vi "log.vi"(8 "error in (no error)":errorcluster, 10 "log_entry":T1 {"datetime" format="%<%x %.3X>T"}, 11 "system.logging.provider in":refnum<class "system.logging.provider.lvclass">) -> (0 "error out":errorcluster, 3 "system.logging.provider out":refnum<class "system.logging.provider.lvclass">)   [LabVIEW 2021, in "system.logging.provider.lvclass"]
uses:
  system.logging.provider.lvclass
  system.logging/log_entry.ctl
  system.logging/severity.ctl
  system.logging.provider.lvclass/system.logging.provider.ctl
  system.logging/system.logging.lvclass
panel:
  out "log_entry_display":T1 {"datetime" format="%<%x %.3X>T"}
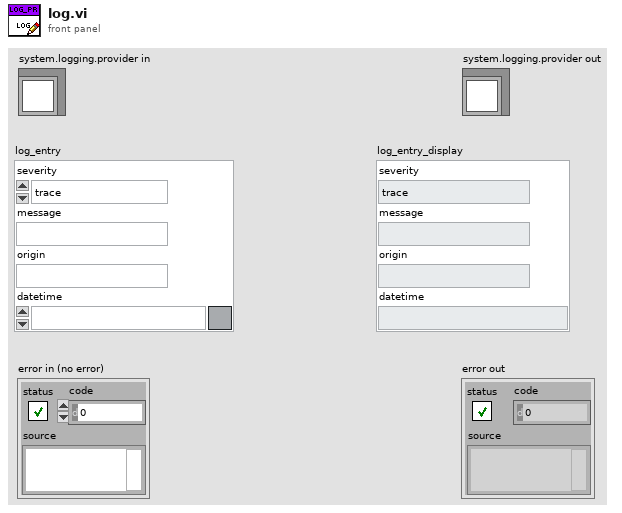
[diagram p1: front panel]
types:
  T1 = typedef "system.logging.lvclass/log_entry.ctl" = cluster{"severity":T2, "message":string, "origin":string, "datetime":timestamp}
  T2 = typedef "system.logging.lvclass/severity.ctl" = enum8{"trace", "debug", "info", "warning", "error"}
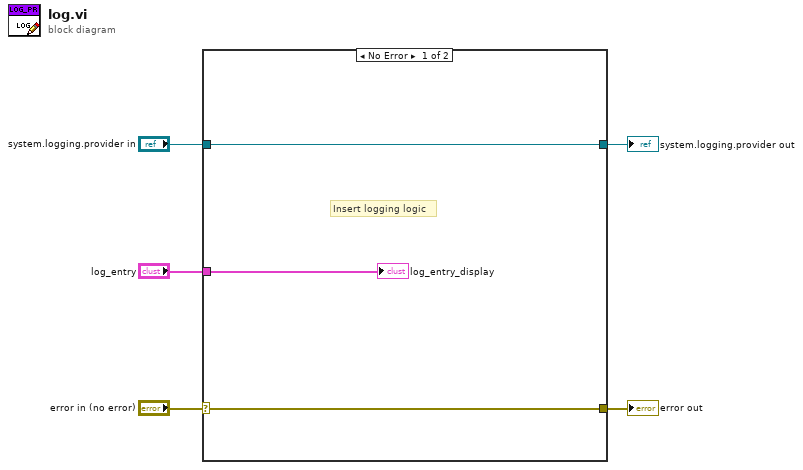
[diagram p0: block diagram]
diagram:
  n1 = case shown="No Error" "error in (no error)" {
    selector: "error in (no error)" -> [w7 w10]
    tunnel: [w7 w10] -> w4
    tunnel: [w6 w9] -> w2
    tunnel: "system.logging.provider in" -> [w6 w9]
    tunnel: "log_entry" -> [w8 _]
    frame No Error {
      # "Insert logging logic"
      "log_entry_display" <- w8
    }
    frame Error {
    }
  }
  "error out" <- w4
  "system.logging.provider out" <- w2
